vi "ShowCommandLineParams.vi"() -> ()   [LabVIEW 2015]
panel:
  out "Application:Command Line Arguments":string[](array[string])
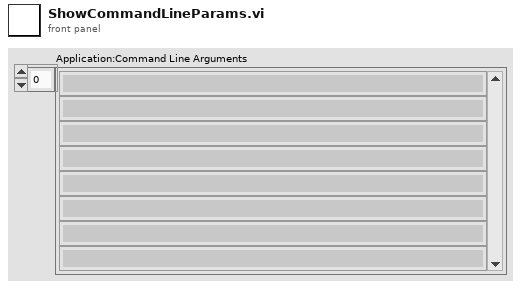
[diagram p1: front panel]
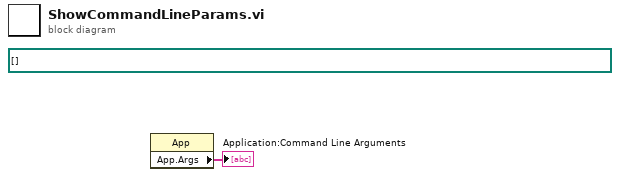
[diagram p0: block diagram]
diagram:
  (unwired) path[] []
  n1 = property class="App"() -> ("App.Args"=→"Application:Command Line Arguments":string[])  [unwired: 2 in, 2 out]
